vi "Handle Response.vi"(7 "Processing In":refnum<class "Processing.lvclass">, 11 "FileExistChecker in":refnum<class "FileExistChecker.lvclass">) -> (0 "error out":errorcluster, 5 "Processing":refnum<class "Processing.lvclass">)   [LabVIEW 2020, in "HTTP Server.lvlib" / "FileExistChecker.lvclass"]
uses:
  FileExistChecker.lvclass
  Processing/Processing.lvclass
  lv-http-util/HTTP Utils/File Response/File Response.lvclass
  Processing/Processing.lvclass/Processing.ctl
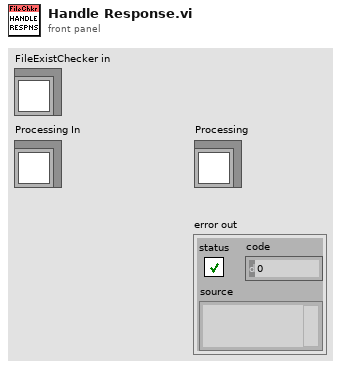
[diagram p1: front panel]
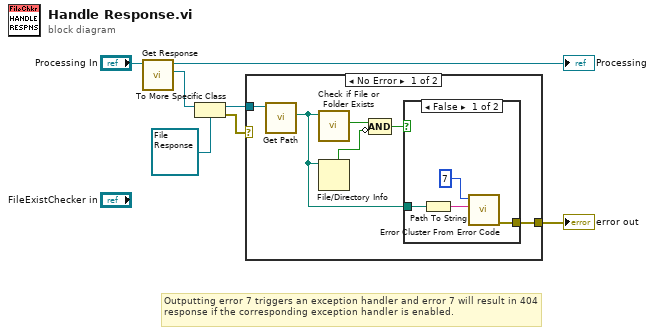
[diagram p0: block diagram]
diagram:
  # "Outputting error 7 triggers an exception handler and error 7 will result in 404 response if the corresponding exception handler is enabled."
  n1 = call "Get Response.vi"("Processing in"="Processing In") -> ("Response"=w2:refnum<class "Response.lvclass">, "Processing out"=→"Processing":refnum<class "Processing.lvclass">)  [unwired: 9 in]
  n2 = To More Specific Class(target class=refnum<class "File Response.lvclass"> refnum ("HTTP Utils.lvlib:File Response.lvclass"), reference=w2) -> (specific class reference=w6:refnum<class "File Response.lvclass">, error out=w7:errorcluster)  [unwired: 1 in]
  n3 = case shown="No Error" w7 {
    tunnel: w6 -> [w9 _]
    tunnel: [w12 _] -> w5
    frame No Error {
      n4 = call "Get Path.vi"("File Response in"=w9) -> ("Path"=w8:path)  [unwired: 8 in, 2 out]
      n5 = call <vilib>:"Check if File or Folder Exists.vi"("path"=w8) -> ("file or folder exists?"=w13:bool)  [unwired: 8 in, 2 out]
      n6 = File/Directory Info(path=w8) -> (directory=w10:bool)  [unwired: 1 in, 6 out]
      n7 = Compound Arithmetic op=AND(w13, invert w10) -> (w11:bool)
      n8 = case shown="False" w11 {
        tunnel: w8 -> [w16 _]
        tunnel: [w14 _] -> w12
        frame False {
          n9 = Path To String(path=w16) -> (string=w15:string)
          n10 = call <vilib>:"Error Cluster From Error Code.vi"("error message (\"\")"=w15, "error code (0)"=7) -> ("error out"=w14:errorcluster)  [unwired: 7 in]
        }
        frame True {
        }
      }
    }
    frame Error {
    }
  }
  "error out" <- w5
